vi "VIH HelpGen - Palette - Get Palette Items.vi"(8 "error in":errorcluster, 11 "Palette Path":path) -> (0 "error out":errorcluster, 2 "Items Array":T1[](array[typedef]), 3 "dup Palette Path":path)   [LabVIEW 2014]
doc: "::: VI Helpeks :::\nCopyright (c) 2000-2026 Konstantin Shifershteyn. All rights reserved."
uses:
  VIH HelpGen Typedef - Palette - Item Info Cluster.ctl
  VIH HelpGen Typedef - Palette - Item Type Enum.ctl
panel:
  # "VI Helpeks\nCopyright (c) 2012-2026 Konstantin Shifershteyn"
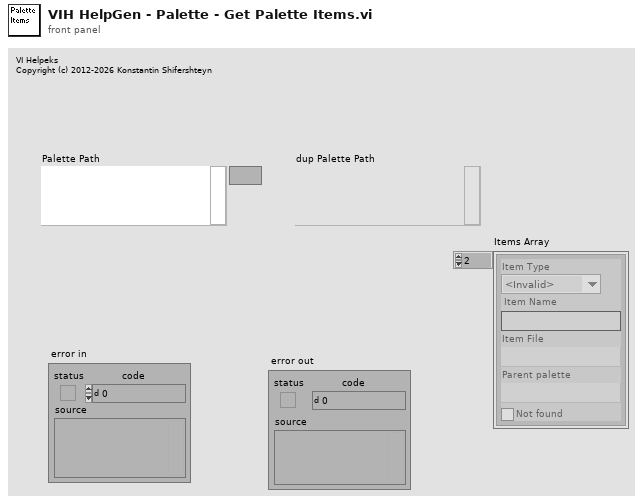
[diagram p1: front panel]
types:
  T1 = typedef "VIH HelpGen Typedef - Palette - Item Info Cluster.ctl" = cluster{"Item Type":T2, "Item Name":string, "Item File":path, "Parent palette":path, "Not found":bool}
  T2 = typedef "VIH HelpGen Typedef - Palette - Item Type Enum.ctl" = enum32{"<Invalid>", "<unknown>", "VI", "Menu", "LV Func", "Express VI", "Poly VI", "CTL", "HTML"}
  T3 = typedef "Palette Menu.lvlib/Palette Data.ctl" = cluster{"display name":string, "view format":T4, "palette width":i16, "items":T5, "256 color icon":picture, "B&W color icon":picture, "help information":T7, "palette description":string, "synchronize information":T8}
  T4 = typedef "Palette Menu.lvlib/View Format.ctl" = u16
  T5 = typedef "Palette Menu.lvlib/Items.ctl" = T6[]
  T6 = typedef "Palette Menu.lvlib/Item.ctl" = cluster{"item path":path, "library path (.lvlib)":path, "use default lvlib palette":bool, "short name":string, "place VI contents":bool, "hide synchronized item":bool, "reserve spot for synch item":bool, "configure when placing VI contents":bool}
  T7 = typedef "Palette Menu.lvlib/Help Info.ctl" = cluster{"help tag":string, "help file path ":path}
  T8 = typedef "Palette Menu.lvlib/Synchronize Info.ctl" = cluster{"synchronize with directory":bool, "synchronize directory path":path}
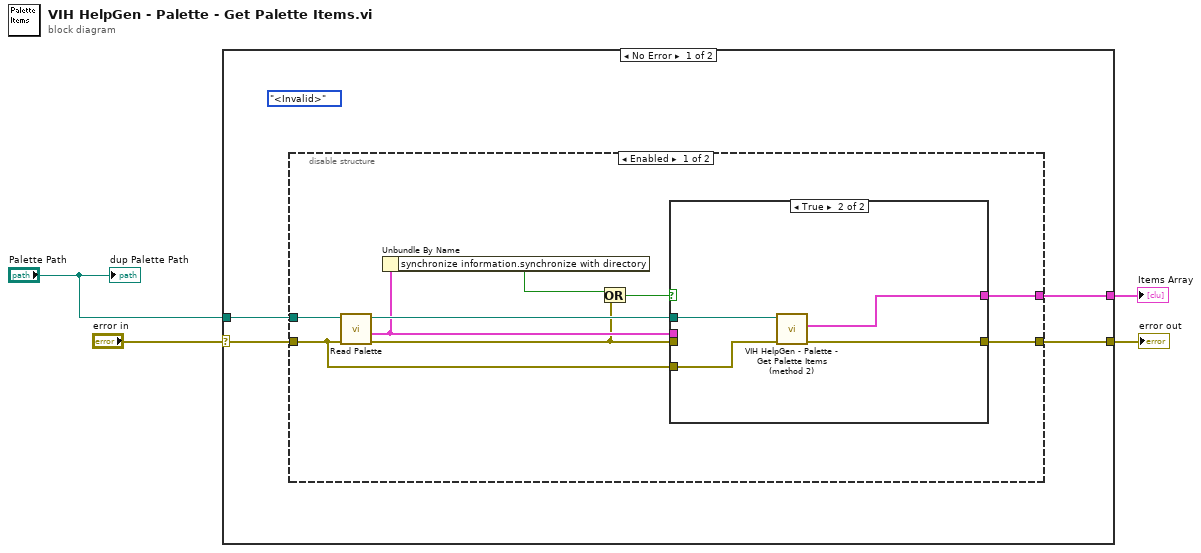
[diagram p0: block diagram]
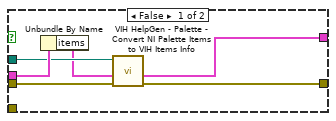
[diagram p2: hidden frame]
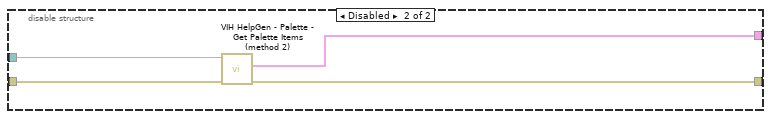
[diagram p3: hidden frame]
diagram:
  n1 = case shown="No Error" "error in" {
    selector: "error in" -> [w5 w32]
    tunnel: "Palette Path" -> [w8 _]
    tunnel: [w7 _] -> w2
    tunnel: [w6 w32] -> w1
    frame No Error {
      (unwired) VIH_HelpGen_Typedef_-_Palette_-_Item_Type_Enum."<Invalid>" ("x")
      n2 = disable-structure shown="Enabled" {
        disable-tunnel: w8 -> [w17 w31]
        disable-tunnel: [w16 w28] -> w7
        disable-tunnel: [w15 w29] -> w6
        disable-tunnel: w5 -> [w14 w30]
        frame Enabled {
          n3 = call <vilib>:"Read Palette.vi"("error in (no error)"=w14, "palette path"=w17) -> ("error out"=w9:errorcluster, "palette data"=w12:T3, "duplicate palette path"=w13:path)  [unwired: 7 in]
          n4 = Unbundle By Name(w12) -> ("synchronize information.synchronize with directory"=w10:bool)
          n5 = Or(x=w10, y=w9) -> (x .or. y?=w11:bool)
          n6 = case shown="True" w11 {
            tunnel: [w18 w26] -> w16
            tunnel: w13 -> [w22 w27]
            tunnel: w12 -> [w23 _]
            tunnel: w9 -> [w20 _]
            tunnel: [w19 w25] -> w15
            tunnel: w14 -> [_ w24]
            frame False {
              n7 = Unbundle By Name(w23) -> ("items"=w21:T5)
              n8 = call "VIH HelpGen - Palette - Convert NI Palette Items to VIH Items Info.vi"("error in"=w20, "Palette Items"=w21, "Palette Path"=w22) -> ("error out"=w19:errorcluster, "Items Array"=w18:T1[])  [unwired: 6 in, 1 out]
            }
            frame True {
              n9 = call "VIH HelpGen - Palette - Get Palette Items (method 2).vi"("error in"=w24, "Palette Path"=w27) -> ("error out"=w25:errorcluster, "Items Array"=w26:T1[])  [unwired: 7 in, 1 out]
            }
          }
        }
        frame Disabled {
          n10 = call "VIH HelpGen - Palette - Get Palette Items (method 2).vi"("error in"=w30, "Palette Path"=w31) -> ("error out"=w29:errorcluster, "Items Array"=w28:T1[])  [unwired: 7 in, 1 out]
        }
      }
    }
    frame Error {
    }
  }
  "Items Array" <- w2
  "error out" <- w1
  "dup Palette Path" <- "Palette Path"
